vi "Burst.vi"(0 "RFFE RegRead Command in":refnum<class "RFFE RegRead Command.lvclass">, 1 "Bus Number":i32, 5 "instrument handle in":refnum<k15>, 11 "error in (no error)":errorcluster) -> (4 "RFFE RegRead Command out":refnum<class "RFFE RegRead Command.lvclass">, 6 "instrument handle out":refnum<k15>, 15 "error out":errorcluster)   [LabVIEW 2018, in "MIPI RFFE API.lvlib" / "RFFE RegRead Command.lvclass"]
uses:
  RFFE RegRead Command.lvclass
  C:/Users/semoore/Projects/mipi-rffe-labview-oop/Standard Command/RFFE Standard Command.lvclass
  Standard Command/RFFE Standard Command.lvclass/RFFE Standard Command.ctl
  RFFE RegRead Command.lvclass/RFFE RegRead Command.ctl
  Standard Command/Set Register Data.vi
  Standard Command/RFFE Standard Command.lvclass
  MIPI RFFE API.lvlib
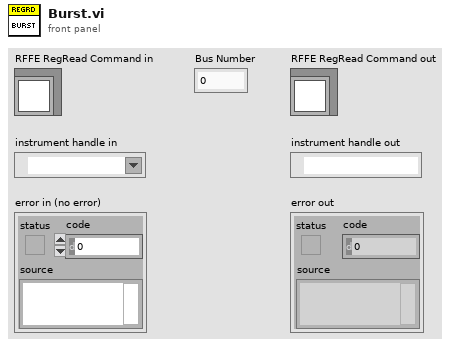
[diagram p1: front panel]
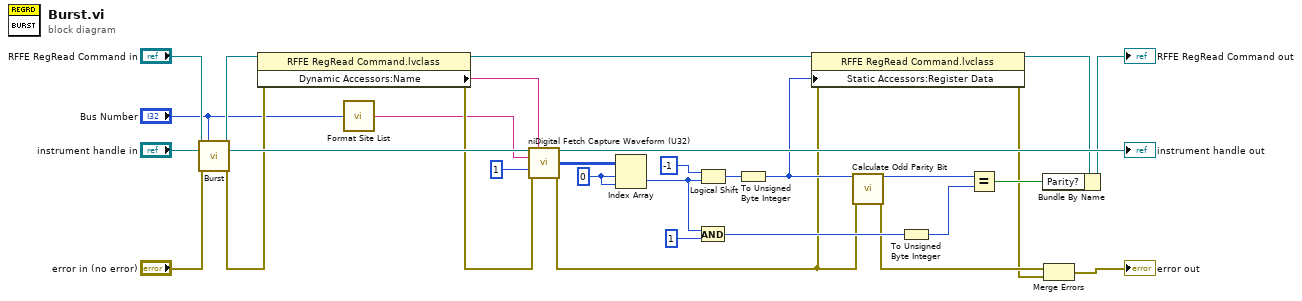
[diagram p0: block diagram]
diagram:
  w17 = 0 ("index (row)")
  n1 = call-parent "Burst.vi"("RFFE Command in"="RFFE RegRead Command in", "Bus Number"="Bus Number", "instrument handle in"="instrument handle in", "error in (no error)"="error in (no error)") -> ("RFFE Command out"=w25:refnum<class "RFFE RegRead Command.lvclass">, "instrument handle out"=w27:refnum<k15>, "error out"=w24:errorcluster)  [unwired: 9 in]
  n2 = property class="RFFE RegRead Command.lvclass"(reference=w25, error in=w24) -> (reference out=w19:refnum<class "RFFE RegRead Command.lvclass">, error out=w21:errorcluster, "Dynamic Accessors:Name"=w22:string)
  n3 = call "Format Site List.vi"("Bus Number"="Bus Number") -> ("Site List"=w16:string)  [unwired: 14 in]
  n4 = call <instrlib>:"niDigital Fetch Capture Waveform (U32).vi"("instrument handle"=w27, "waveform name"=w22, "site list"=w16, "samples to read"=1, "error in"=w21) -> ("instrument handle out"=→"instrument handle out":refnum<k15>, "data"=w18:u32[][], "error out"=w5:errorcluster)  [unwired: 8 in]
  n5 = Index Array(array=w18, index (row)=w17, index (col)=w17) -> (element=w14:u32)
  n6 = Logical Shift(y=i16 -1, x=w14) -> (x << y=w12:u32)
  n7 = And(x=w14, y=u32 1) -> (x .and. y?=w7:u32)
  n8 = To Unsigned Byte Integer(number=w12) -> (unsigned 8bit integer=w11:u8)
  n9 = property class="RFFE RegRead Command.lvclass"(reference=w19, error in=w5, "Static Accessors:Register Data"=w11) -> (reference out=w10:refnum<class "RFFE RegRead Command.lvclass">, error out=w2:errorcluster)
  n10 = call "Calculate Odd Parity Bit.vi"("Byte"=w11, "error in (no error)"=w5) -> ("Odd Parity Bit"=w8:u8, "error out"=w3:errorcluster)  [unwired: 12 in]
  n11 = To Unsigned Byte Integer(number=w7) -> (unsigned 8bit integer=w6:u8)
  n12 = Equal?(x=w8, y=w6) -> (x = y?=w4:bool)
  n13 = Bundle By Name(cluster=w10, "Parity?"=w4) -> (→"RFFE RegRead Command out":refnum<class "RFFE RegRead Command.lvclass">)
  n14 = Merge Errors(w3, w2) -> (→"error out":errorcluster)
